vi "Module Init.vi"(8 "error in (no error)":errorcluster, 11 "Historian Logger in":refnum<class "Historian Logger.lvclass">) -> (0 "error out":errorcluster, 3 "Historian Logger out":refnum<class "Historian Logger.lvclass">)   [LabVIEW 2020, in "VolatusHistorian.lvlib" / "Historian Logger.lvclass"]
uses:
  Historian Logger.lvclass
  Historian Logger.lvclass/Historian Logger.ctl
  Volatus/Module/Module.lvclass
  C:/dev/lv20CE/relink/lv-volatus/Volatus/Module/Module.lvclass
  C:/dev/lv20CE/relink/lv-volatus/VolatusHistorian/Historian Logger/Historian Logger.lvclass
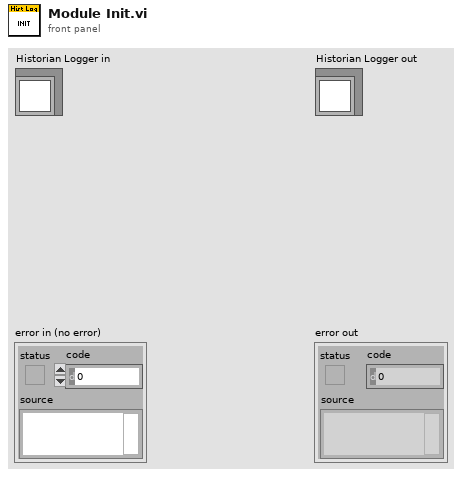
[diagram p1: front panel]
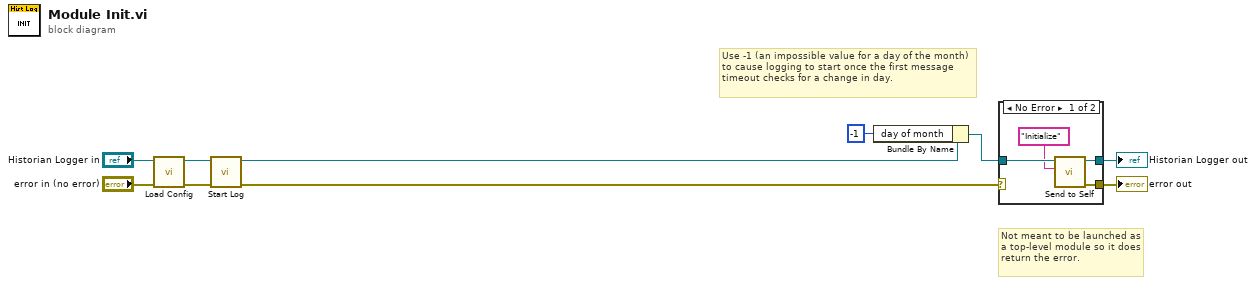
[diagram p0: block diagram]
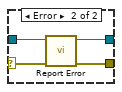
[diagram p2: hidden frame]
diagram:
  # "Use -1 (an impossible value for a day of the month) to cause logging to start once the first message timeout checks for a change in day."
  # "Not meant to be launched as a top-level module so it does return the error."
  n1 = call "Load Config.vi"("error in (no error)"="error in (no error)", "Historian Logger in"="Historian Logger in") -> ("error out"=w7:errorcluster, "Historian Logger out"=w4:refnum<class "Historian Logger.lvclass">)  [unwired: 8 in]
  n2 = call "Start Log.vi"("error in (no error)"=w7, "Historian Logger in"=w4) -> ("error out"=w5:errorcluster, "Historian Logger out"=w3:refnum<class "Historian Logger.lvclass">)  [unwired: 8 in]
  n3 = Bundle By Name(cluster=w3, "day of month"=-1) -> (w2:refnum<class "Historian Logger.lvclass">)
  n4 = case shown="No Error" w5 {
    selector: w5 -> [_ w17]
    tunnel: [w14 w15] -> w9
    tunnel: w2 -> [w13 w18]
    tunnel: [w12 w16] -> w8
    frame No Error {
      n5 = call "Send to Self.vi"("Message ID"="Initialize", "Module in"=w13) -> ("error out"=w14:errorcluster, "Module out"=w12:refnum<class "Historian Logger.lvclass">)  [unwired: 8 in]
    }
    frame Error {
      n6 = call "Report Error.vi"("error in (no error)"=w17, "Module in"=w18) -> ("error out"=w15:errorcluster, "Module out"=w16:refnum<class "Historian Logger.lvclass">)  [unwired: 8 in]
    }
  }
  "error out" <- w9
  "Historian Logger out" <- w8
